vi "CSE - Diagnose Script.vi"(6 "sort (F)":bool, 8 "error in":errorcluster, 9 "Items":i32(ring) items=["Variables", "Functions", "FuncVI functions", "FastFunc functions"], 11 "CSE RefNum":T1) -> (0 "error out":errorcluster, 1 "Array of Items":string[](array[string]), 3 "dup CSE RefNum":T1)   [LabVIEW 2021]
doc: "This VI returns the names of variables and functions referenced in a parsed script. Refer to the VI help for more details.\n\n::: CalcExpress Toolkit :::\nCopyright (c) 2000-2026 Konstantin Shifershteyn. All rights reserved."
uses:
  CSE Instance RefNum.ctl
  cersrc/celveng32.dll
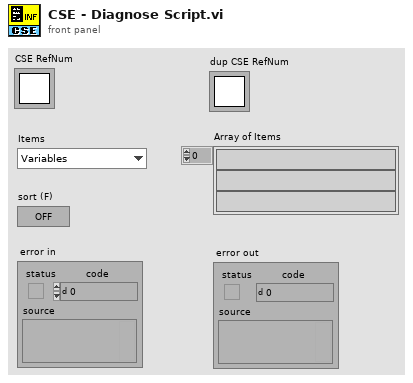
[diagram p1: front panel]
types:
  T1 = typedef "CSE Instance RefNum.ctl" = refnum<k1>
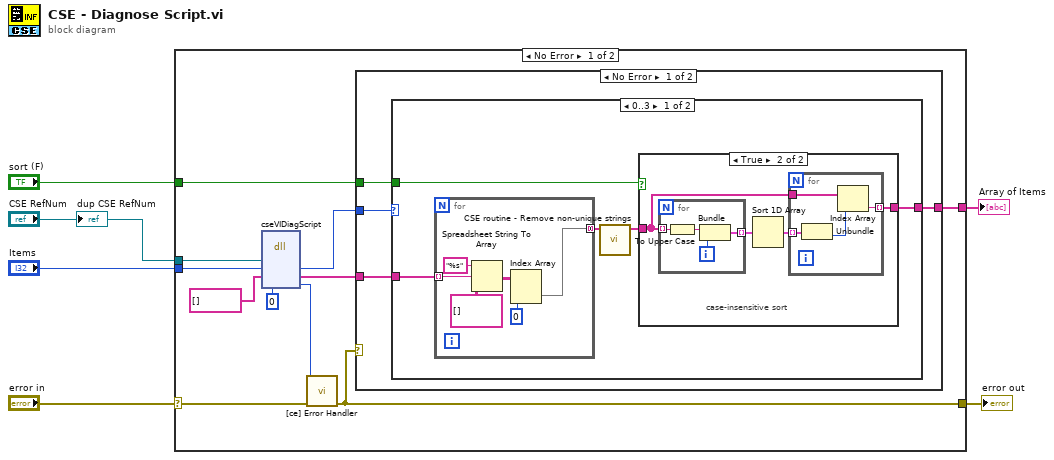
[diagram p0: block diagram]
diagram:
  n1 = case shown="No Error" "error in" {
    selector: "error in" -> [w13 w47]
    tunnel: "CSE RefNum" -> [w17 _]
    tunnel: [w12 w47] -> w4
    tunnel: "Items" -> [w16 _]
    tunnel: [w10 _] -> w2
    tunnel: "sort (F)" -> [w9 _]
    frame No Error {
      n2 = dll-call lib="C:/LV Projects/CalcExpress 40 LV2021/vi.lib/addons/CalcExpress/cersrc/celveng*.dll" fn="cseVIDiagScript"("iCESP"=w17, "ItemID"=w16, "ArrOfStr"=string[] [] ("Array of Items"), "errStat"=0) -> ("ItemID"=w7:i32, "ArrOfStr"=w11:string[], "errStat"=w14:i32)  [unwired: 5 in, 2 out]
      n3 = call "[ce] Error Handler.vi"("error in"=w13, "error code"=w14) -> ("error out"=w12:errorcluster)  [unwired: 8 in, 1 out]
      n4 = case shown="No Error" w12 {
        tunnel: w11 -> [w21 _]
        tunnel: [w20 _] -> w10
        tunnel: w9 -> [w19 _]
        tunnel: w7 -> [w18 _]
        frame No Error {
          n5 = case shown="0..3" w18 {
            tunnel: w21 -> [w26 w46]
            tunnel: [w24 w46] -> w20
            tunnel: w19 -> [w23 _]
            frame 0..3 {
              n6 = for {
                tunnel: w26 -> [w41] mode=indexing
                tunnel: [w40] -> w22 mode=concatenating
                n7 = Spreadsheet String To Array(format string="%s", spreadsheet string=w41, array type (2D Dbl)=string[][] []) -> (array=w43:string[][])  [unwired: 1 in]
                n8 = Index Array(array=w43, index (col)=0 ("disabled index (col)")) -> (element=w40:string[])  [unwired: 1 in]
              }
              n9 = call "CSE routine - Remove non-unique strings.vi"("Array in"=w22) -> ("Array out"=w25:string[])  [unwired: 7 in, 1 out]
              n10 = case shown="True" w23 {
                tunnel: w25 -> [w27 w29]
                tunnel: [w27 w28] -> w24
                frame False {
                }
                frame True {
                  # "case-insensitive sort"
                  n11 = for {
                    tunnel: w29 -> [w38] mode=indexing
                    tunnel: [w36] -> w31 mode=indexing
                    i -> [w39]
                    n12 = To Upper Case(1:w38) -> (0:w37:string)
                    n13 = Bundle(w37, w39) -> (w36:cluster{string, i32})  [unwired: 1 in]
                  }
                  n14 = Sort 1D Array(array=w31) -> (sorted array=w30:cluster{string, i32}[])
                  n15 = for {
                    tunnel: w30 -> [w35] mode=indexing
                    tunnel: w29 -> [w34]
                    tunnel: [w32] -> w28 mode=indexing
                    n16 = Unbundle(w35) -> (w33:i32)  [unwired: 1 out]
                    n17 = Index Array(array=w34, index=w33) -> (element=w32:string)
                  }
                }
              }
            }
            frame Default {
            }
          }
        }
        frame Error {
        }
      }
    }
    frame Error {
    }
  }
  "error out" <- w4
  "Array of Items" <- w2
  "dup CSE RefNum" <- "CSE RefNum"
